vi "Localize This VI.vi"   [LabVIEW 2017]
uses:
  API/JKI Simple Localization.lvlib
types:
  T1 = enum32{"invalid OS target", "Mac OS", "Windows 3.1", "Windows 95/NT", "Solaris 1", "Solaris 2", "HP-UX", "PowerMAX", "Linux", "Irix", "Rhapsody", "BeOS", "AIX", "OSF1", "VxWorks", "PharLap", "Carbon", "RTX", "Windows x64", "Linux x64", "Mac OS X x64"}
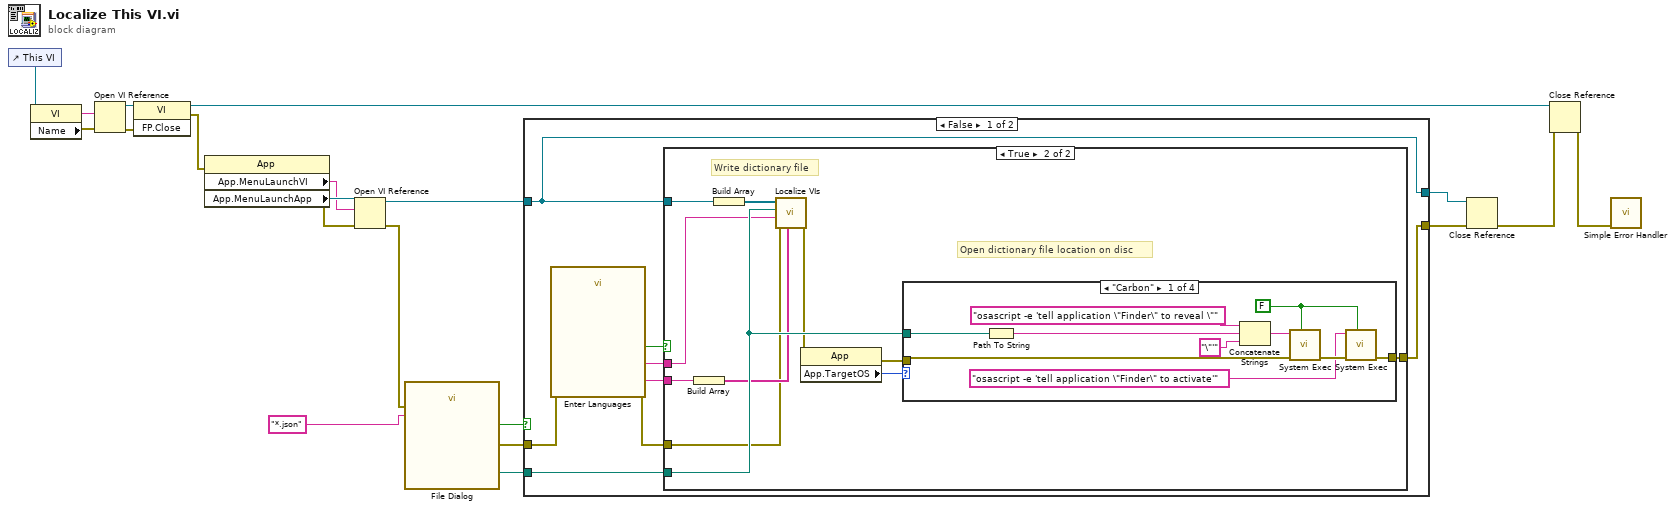
[diagram p0: block diagram]
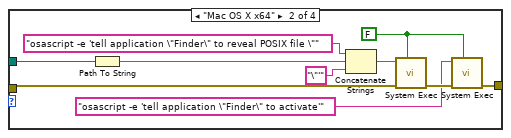
[diagram p3: hidden frame]
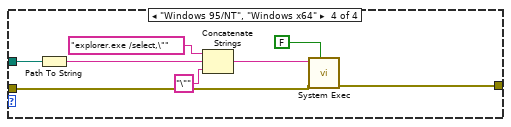
[diagram p5: hidden frame]
diagram:
  n1 = control-ref of="This VI"() -> (w16:refnum<vi>)
  n2 = property class="VI"(reference=w16) -> (error out=w12:errorcluster, "Name"=w15:string)  [unwired: 1 in, 1 out]
  n3 = Open VI Reference(vi path=w15, error in (no error)=w12) -> (vi reference=w14:refnum<vi>, error out=w11:errorcluster)  [unwired: 4 in]
  n4 = invoke class="VI" method="FP.Close"(reference=w14, error in=w11) -> (reference out=w10:refnum<vi>, error out=w13:errorcluster)  [unwired: 1 in, 1 out]
  n5 = property class="App"(error in=w13) -> (error out=w18:errorcluster, "App.MenuLaunchVI"=w19:string, "App.MenuLaunchApp"=w20:refnum<vi>)  [unwired: 1 in, 1 out]
  n6 = Open VI Reference(application reference (local)=w20, vi path=w19, error in (no error)=w18) -> (vi reference=w8:refnum<vi>, error out=w17:errorcluster)  [unwired: 3 in]
  n7 = call "File Dialog"("error in"=w17, "pattern (all files)"="*.json" ("pattern label")) -> ("selected path"=w6:path, "cancelled"=w4:bool, "error out"=w5:errorcluster)  [unwired: 10 in, 1 out]
  n8 = case shown="False" w4 {
    tunnel: w8 -> [w28 w71]
    tunnel: w6 -> [w27 _]
    tunnel: w5 -> [w23 w70]
    tunnel: [w28 w71] -> w3
    tunnel: [w26 w70] -> w2
    frame False {
      n9 = call "Enter Languages"("error in (no error)"=w23) -> ("Additional Language"=w24:string, "Current Language"=w25:string, "OK"=w21:bool, "error out"=w22:errorcluster)  [unwired: 15 in]
      n10 = case shown="True" w21 {
        tunnel: w28 -> [_ w39]
        tunnel: w27 -> [_ w37]
        tunnel: [w29 w34] -> w26
        tunnel: w25 -> [_ w33]
        tunnel: w24 -> [_ w32]
        tunnel: w22 -> [w29 w30]
        frame False {
        }
        frame True {
          # "Open dictionary file location on disc"
          # "Write dictionary file"
          n11 = Build Array(w32) -> (w31:string[])
          n12 = Build Array(w39) -> (w40:refnum<vi>[])
          n13 = call "Localize VIs.vi"("Additional Languages [English]"=w31, "error in (no error)"=w30, "Current VI Language (English)"=w33, "Dictionary Path"=w37, "VIs in"=w40) -> ("error out"=w36:errorcluster)  [unwired: 6 in]
          n14 = property class="App"(error in=w36) -> (error out=w35:errorcluster, "App.TargetOS"=w38:T1)  [unwired: 1 in, 1 out]
          n15 = case shown="\"Carbon\"" w38 {
            tunnel: w37 -> [w43 w55 _ w65]
            tunnel: w35 -> [w41 w51 w61 w63]
            tunnel: [w42 w52 w61 w62] -> w34
            frame "Carbon" {
              w46 = FALSE ("wait until completion? (T)")
              n16 = Path To String(path=w43) -> (string=w44:string)
              n17 = Concatenate Strings("osascript -e 'tell application \"Finder\" to reveal \"" ("string"), w44, "\"'" ("string")) -> (w48:string)
              n18 = call <vilib>:"System Exec.vi"("wait until completion? (T)"=w46, "error in (no error)"=w41, "command line"=w48) -> ("error out"=w47:errorcluster)  [unwired: 5 in, 3 out]
              n19 = call <vilib>:"System Exec.vi"("wait until completion? (T)"=w46, "error in (no error)"=w47, "command line"="osascript -e 'tell application \"Finder\" to activate'" ("string")) -> ("error out"=w42:errorcluster)  [unwired: 5 in, 3 out]
            }
            frame "Mac OS X x64" {
              w57 = FALSE ("wait until completion? (T)")
              n20 = Path To String(path=w55) -> (string=w54:string)
              n21 = Concatenate Strings("osascript -e 'tell application \"Finder\" to reveal POSIX file \"" ("string"), w54, "\"'" ("string")) -> (w59:string)
              n22 = call <vilib>:"System Exec.vi"("wait until completion? (T)"=w57, "error in (no error)"=w51, "command line"=w59) -> ("error out"=w58:errorcluster)  [unwired: 5 in, 3 out]
              n23 = call <vilib>:"System Exec.vi"("wait until completion? (T)"=w57, "error in (no error)"=w58, "command line"="osascript -e 'tell application \"Finder\" to activate'" ("string")) -> ("error out"=w52:errorcluster)  [unwired: 5 in, 3 out]
            }
            frame Default {
            }
            frame "Windows 95/NT", "Windows x64" {
              n24 = Path To String(path=w65) -> (string=w64:string)
              n25 = Concatenate Strings("explorer.exe /select,\"" ("string"), w64, "\"" ("string")) -> (w67:string)
              n26 = call <vilib>:"System Exec.vi"("wait until completion? (T)"=FALSE, "error in (no error)"=w63, "command line"=w67) -> ("error out"=w62:errorcluster)  [unwired: 5 in, 3 out]
            }
          }
        }
      }
    }
    frame True {
    }
  }
  n27 = Close Reference(reference=w3, error in (no error)=w2) -> (error out=w7:errorcluster)
  n28 = Close Reference(reference=w10, error in (no error)=w7) -> (error out=w9:errorcluster)
  n29 = call <vilib>:"Simple Error Handler.vi"("error in (no error)"=w9) -> ()  [unwired: 4 in, 5 out]
